vi "Dialog_TGC (SubVI).vi"() -> ()   [LabVIEW 2017]
uses:
  Control_EU/AScanXY.ctl
  Global_SNK3_HF.vi
panel:
  out "Array":dbl[](array[numeric])
  out "output array":dbl[](array[numeric])
  in  "Tab Control":T1(tab)
  out "DACTbl":dbl[][](array[numeric])
  out "TGC_Tbl":dbl[][](array[numeric])
  out "TGCTbl":dbl[][](array[numeric])=[[7.843137254901963e-08, 1.0457516339869285e-06, 2.1960784313725495e-06, 3.2941176470588244e-06, 4.078431372549021e-06, 4.993464052287583e-06, 5.725490196078433e-06, 7.686274509803923e-06, 8e-06], [0.039867986798679866, 0.030858085808580876, 0.036006600660066, 0.032574257425742575, 0.03900990099009902, 0.039438943894389455, 0.0282838283828383, 0.023993399339933996, 8e-06], [0.0, 1e-06, 2e-06, 3e-06, 4e-06, 5e-06, 6e-06, 7e-06, 8e-06], [0.0, 1e-06, 2e-06, 3e-06, 4e-06, 5e-06, 6e-06, 7e-06, 8e-06], [0.0, 1e-06, 2e-06, 3e-06, 4e-06, 5e-06, 6e-06, 7e-06, 8e-06], [0.0, 1e-06, 2e-06, 3e-06, 4e-06, 5e-06, 6e-06, 7e-06, 8e-06], [0.0, 1e-06, 2e-06, 3e-06, 4e-06, 5e-06, 6e-06, 7e-06, 8e-06], [0.0, 1e-06, 2e-06, 3e-06, 4e-06, 5e-06, 6e-06, 7e-06, 8e-06]]
  out "CurTbl":dbl[][](array[numeric])=[[7.843137254901963e-08, 1.0457516339869285e-06, 2.1960784313725495e-06, 3.2941176470588244e-06, 4.078431372549021e-06, 4.993464052287583e-06, 5.725490196078433e-06, 7.686274509803923e-06, 8e-06], [0.039867986798679866, 0.030858085808580876, 0.036006600660066, 0.032574257425742575, 0.03900990099009902, 0.039438943894389455, 0.0282838283828383, 0.023993399339933996, 8e-06], [0.0, 1e-06, 2e-06, 3e-06, 4e-06, 5e-06, 6e-06, 7e-06, 8e-06], [0.0, 1e-06, 2e-06, 3e-06, 4e-06, 5e-06, 6e-06, 7e-06, 8e-06], [0.0, 1e-06, 2e-06, 3e-06, 4e-06, 5e-06, 6e-06, 7e-06, 8e-06], [0.0, 1e-06, 2e-06, 3e-06, 4e-06, 5e-06, 6e-06, 7e-06, 8e-06], [0.0, 1e-06, 2e-06, 3e-06, 4e-06, 5e-06, 6e-06, 7e-06, 8e-06], [0.0, 1e-06, 2e-06, 3e-06, 4e-06, 5e-06, 6e-06, 7e-06, 8e-06]]
  in  "y":dbl=64.0 format="%#_13g"
  in  "Log":refnum<vi>
  in  "WrtTGC":bool
  in  "Tick":T2(ring)
  in  "ВРЧ":string[][](table)
  in  "Stop":bool
  out "TGCGraph":T3 caption="XY Graph - Light"
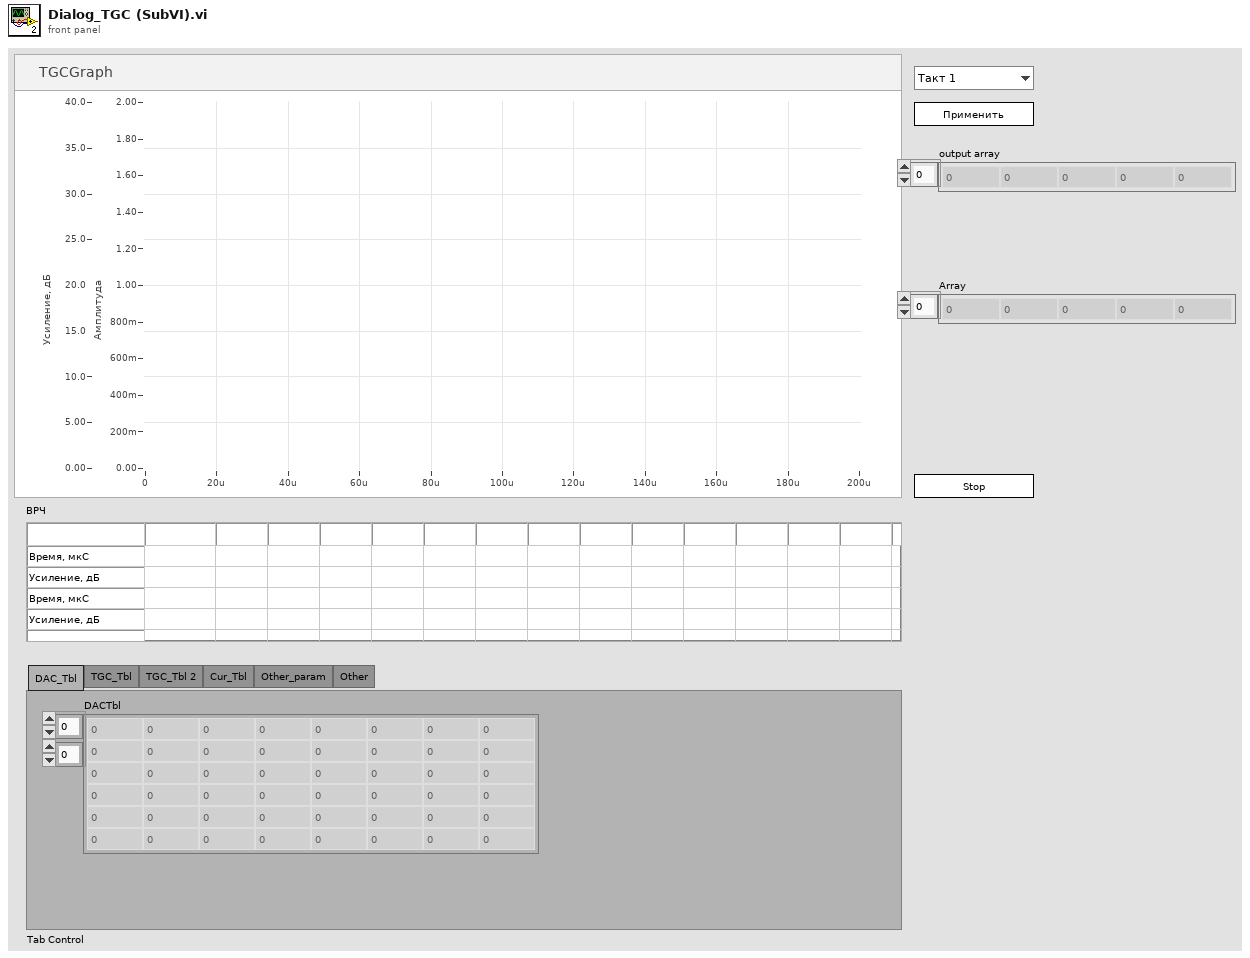
[diagram p1: front panel]
types:
  T1 = enum32{"DAC_Tbl", "TGC_Tbl", "TGC_Tbl 2", "Cur_Tbl", "Other_param", "Other"}
  T2 = enum16{"Такт 1", "Такт 2", "Такт 3", "Такт 4", "Такт 5", "Такт 6", "Такт 7", "Такт 8", "Такт 9", "Такт 10", "Такт 11", "Такт 12", "Такт 13", "Такт 14", "Такт 15", "Такт 16", "Такт 17", "Такт 18", "Такт 19", "Такт 20", "Такт 21", "Такт 22", "Такт 23", "Такт 24", "Такт 25", "Такт 26", "Такт 27", "Такт 28", "Такт 29", "Такт 30", "Такт 31", "Такт 32"}
  T3 = typedef "AScanXY.ctl" = cluster{dbl[], dbl[]}[]
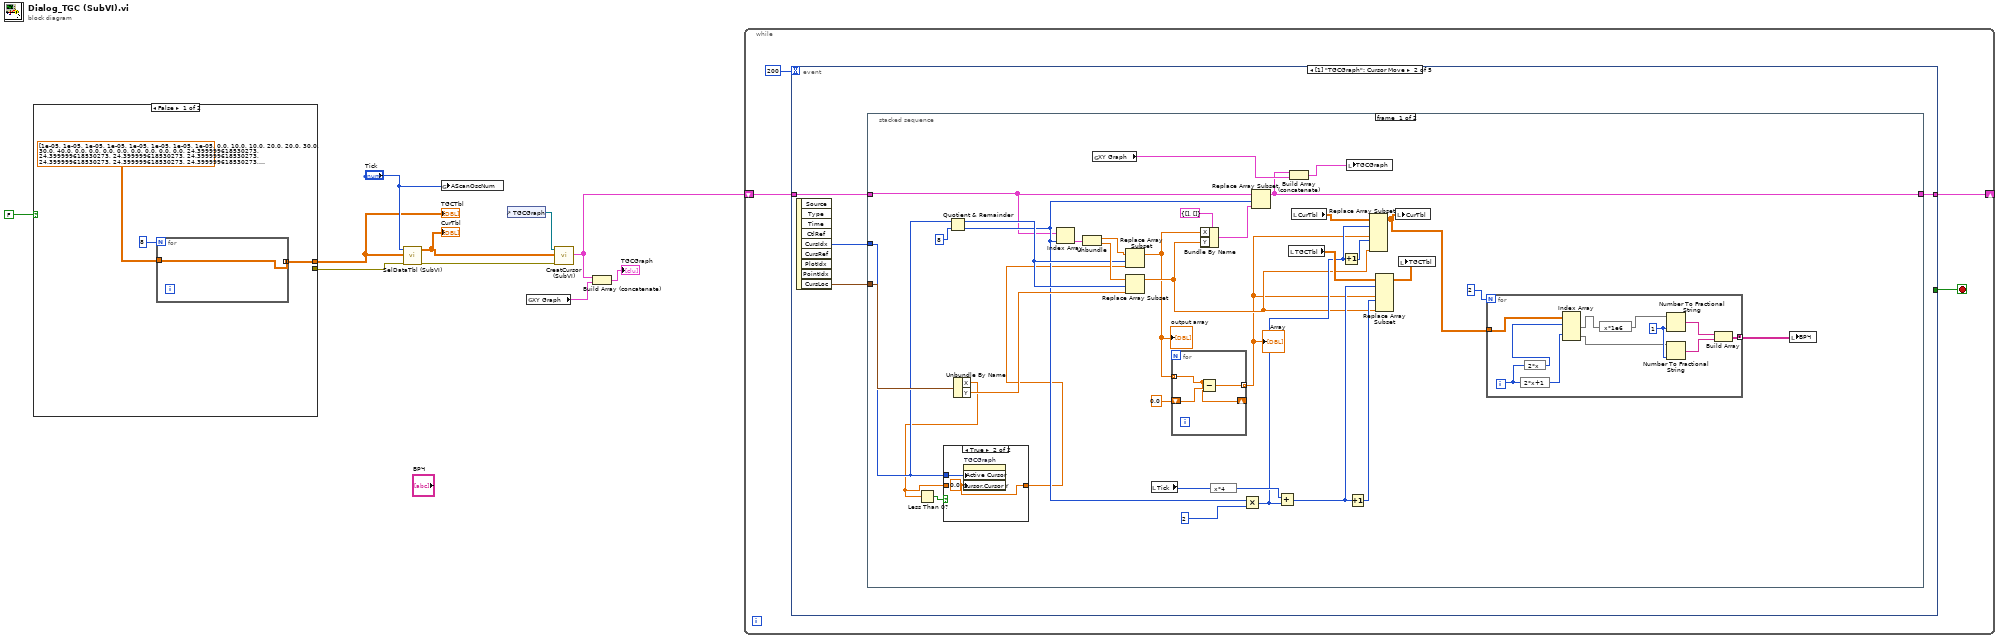
[diagram p0: block diagram]
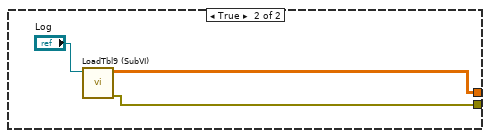
[diagram p2: hidden frame]
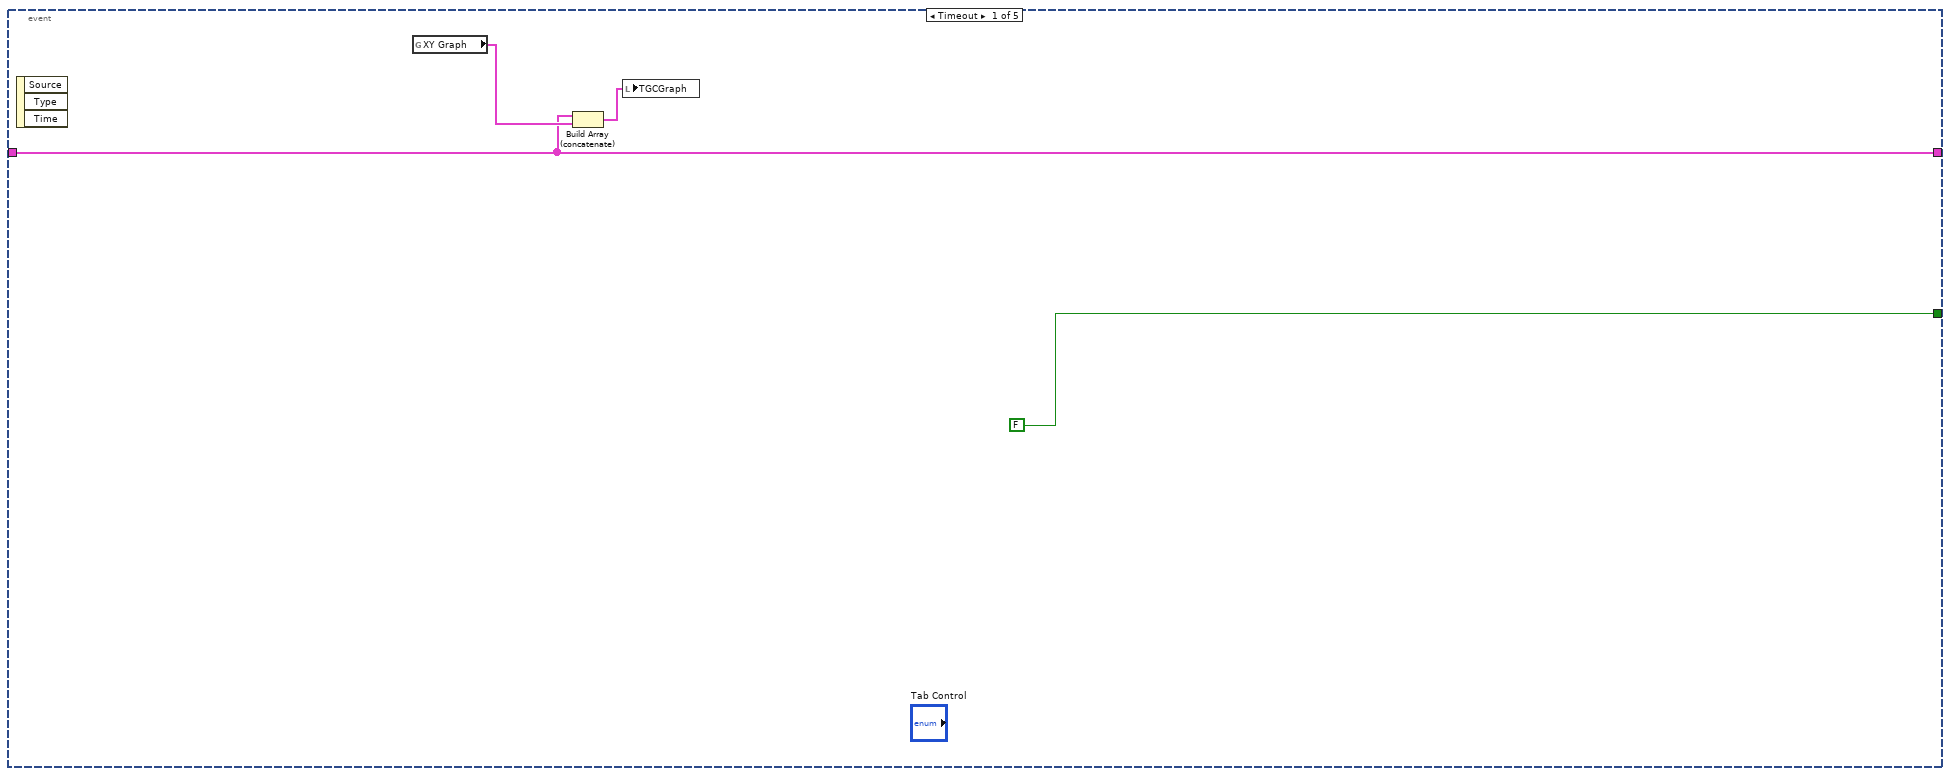
[diagram p3: hidden frame]
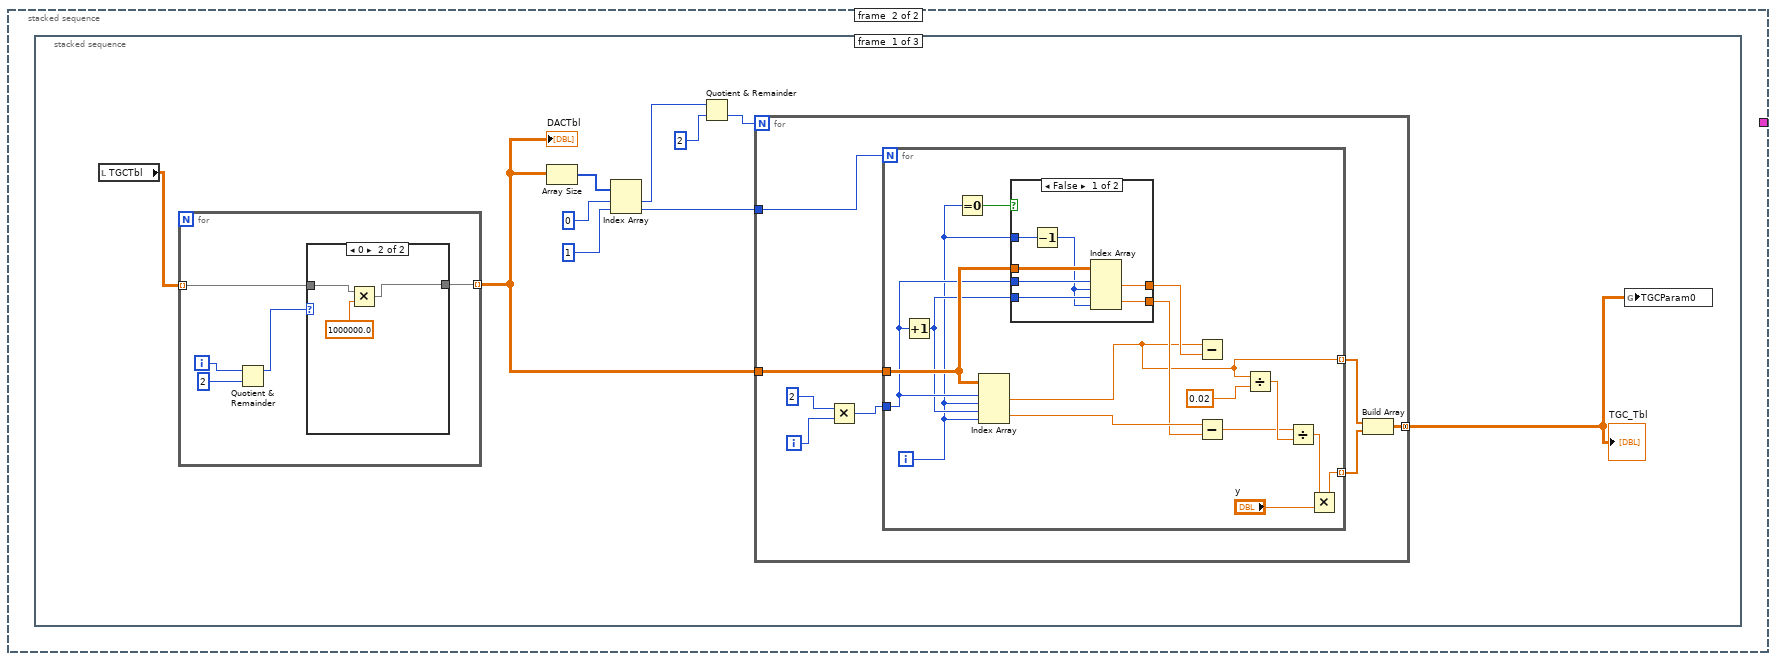
[diagram p5: hidden frame]
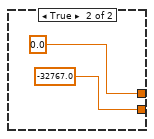
[diagram p6: hidden frame]
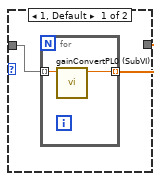
[diagram p7: hidden frame]
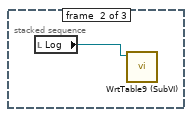
[diagram p8: hidden frame]
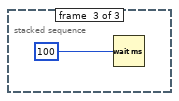
[diagram p9: hidden frame]
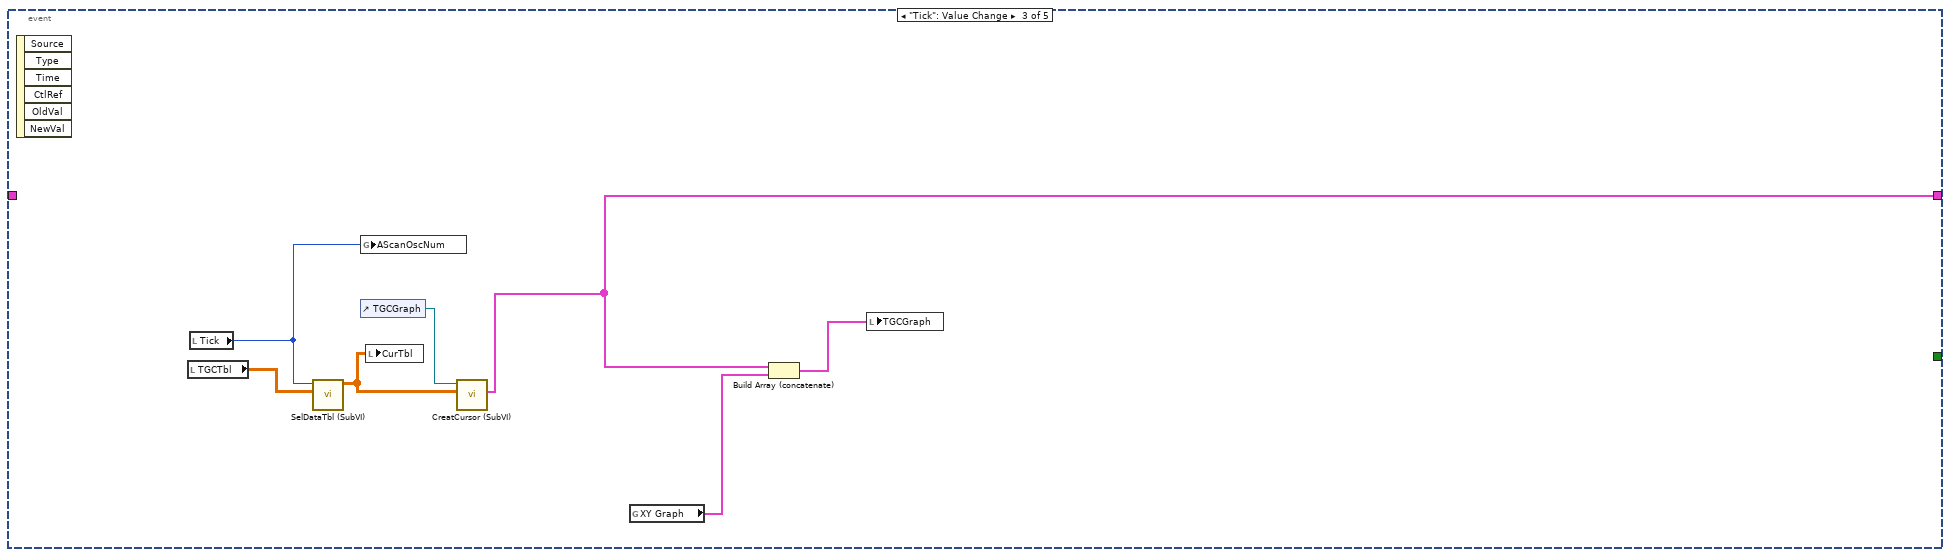
[diagram p10: hidden frame]
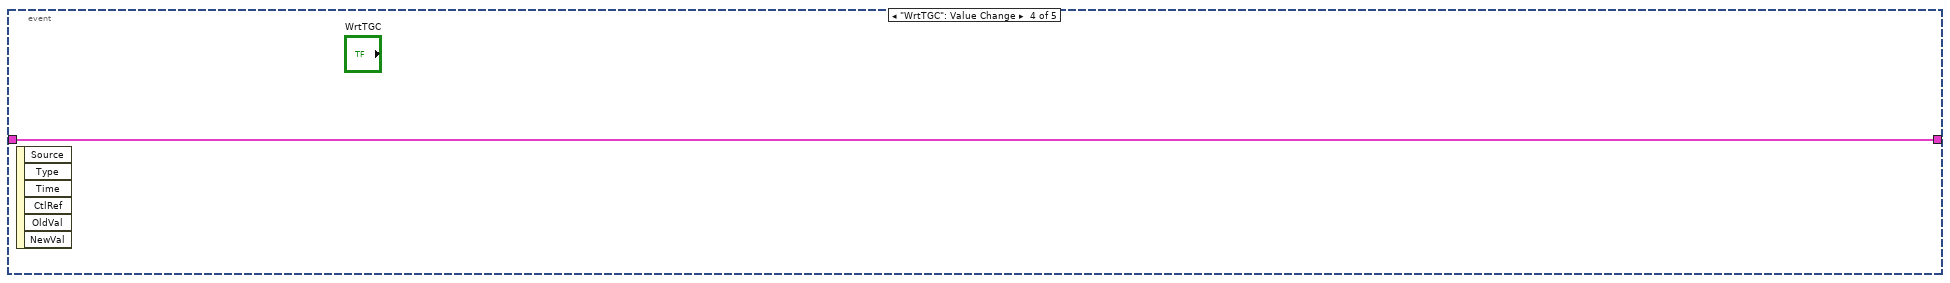
[diagram p11: hidden frame]
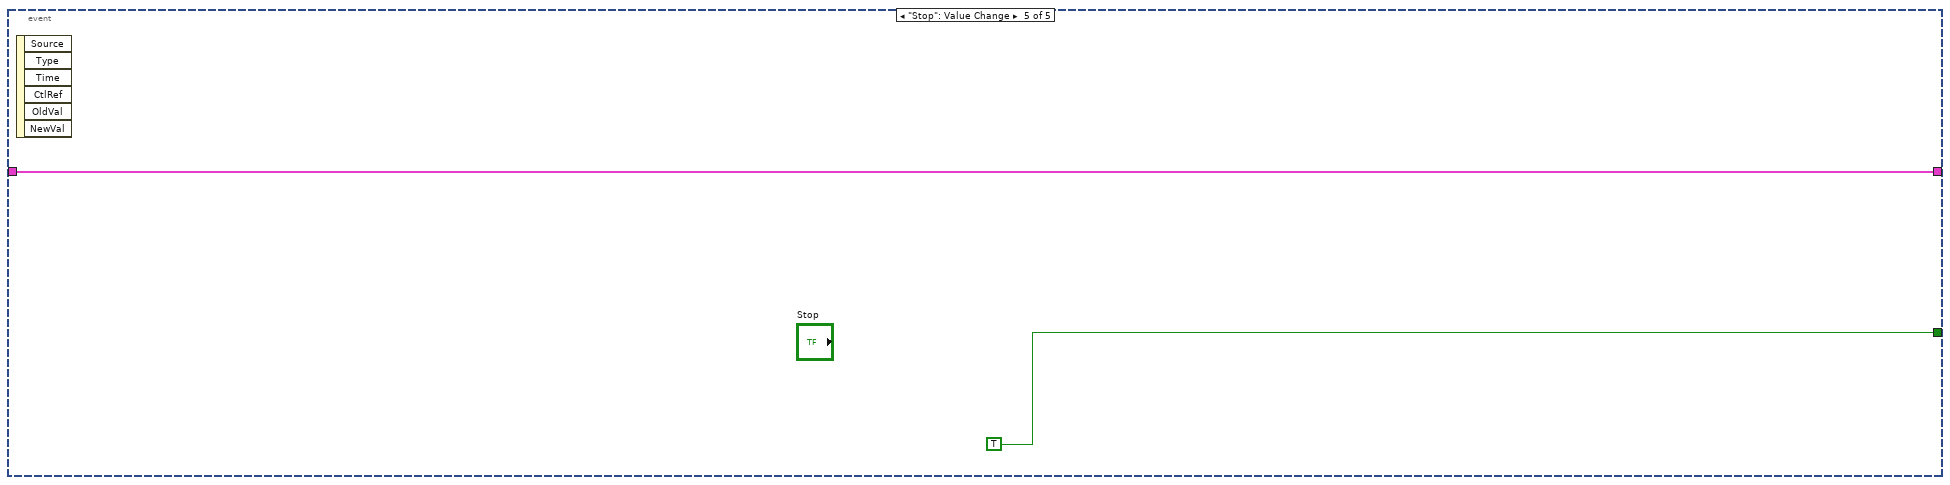
[diagram p12: hidden frame]
diagram:
  n1 = case shown="False" FALSE {
    tunnel: [w12 w16] -> w2
    tunnel: [_ w15] -> w1
    frame False {
      n2 = for {
        N: 8 -> [_]
        tunnel: [w14] -> w12 mode=concatenating
        tunnel: dbl[][] [[1e-05, 1e-05, 1e-05, 1e-05, 1e-05, 1e-05, 1e-05, 1e-05], [0.0, 10.0, 10.0, 20.0, 20.0, 30.0, 30.0, 40.0], [0.0, 0.0, 0.0, 0.0, 0.0, 0.0, 0.0, 0.0], [24.399999618530273, 24.399999618530273, 24.399999618530273, 24.399999618530273, 24.399999618530273, 24.399999618530273, 24.399999618530273, 24.399999618530273]] ("CurTbl 2") -> [w14]
      }
    }
    frame True {
      n3 = call "LoadTbl9 (SubVI).vi"("Log"="Log") -> ("error out"=w15:errorcluster, "Array"=w16:sgl[][])  [unwired: 9 in]
    }
  }
  "TGCTbl" <- w2
  n4 = call "SelDataTbl (SubVI).vi"("error in (no error)"=w1, "In"=w2, "Enum"="Tick") -> ("error out"=w4:errorcluster, "Out"=w3:dbl[][])  [unwired: 7 in]
  "CurTbl" <- w3
  n5 = global write "Global_SNK3_HF.vi" "AScanOscNum"("Tick") -> ()
  n6 = control-ref of="TGCGraph"() -> (w7:refnum<vi>)
  n7 = global read "Global_SNK3_HF.vi" "XY Graph"() -> (w10:cluster{dbl[], dbl[]})
  n8 = call "CreatCursor (SubVI).vi"("error in (no error)"=w4, "Array in"=w3, "XYGraph in"=w7) -> ("Array out"=w8:cluster{"X":dbl[], "Y":dbl[]}[])  [unwired: 8 in]
  n9 = Build Array (concatenate)(w8, w10) -> (→"TGCGraph":cluster{"X":dbl[], "Y":dbl[]}[])
  n10 = while {
    shift-right: [w19] -> _
    shift-left: w8 -> [w18]
    stop <- w21 stop-if-true
    n11 = event shown="[1] \"TGCGraph\": Cursor Move" {
      selector: _ -> [_ _ _ _ _]
      dyn-events: _ -> [_ _ _ _ _]
      timeout: 200 -> [_ _ _ _ _]
      tunnel: [FALSE _ _ _ TRUE] -> w21
      tunnel: w18 -> [w22 w27 _ w145 w146]
      tunnel: [w22 w28 w139 w145 w146] -> w19
      event Timeout {
        n12 = event-data() -> ()  [unwired: 1 in, 3 out]
        n13 = global read "Global_SNK3_HF.vi" "XY Graph"() -> (w24:cluster{dbl[], dbl[]})
        n14 = Build Array (concatenate)(w22, w24) -> (w23:cluster{"X":dbl[], "Y":dbl[]}[])
        n15 = local write "TGCGraph"(w23) -> ()
      }
      event Cursor Move {
        n16 = event-data() -> ("CursIdx"=w26:i32, "CursLoc"=w29:cluster{"X":dbl, "Y":dbl})  [unwired: 1 in, 7 out]
        n17 = stacked-sequence {
          tunnel: w29 -> [w64 _]
          tunnel: [w50 _] -> w28
          tunnel: w27 -> [w49 _]
          tunnel: w26 -> [w47 _]
          frame #0 {
            n18 = Quotient & Remainder(x=w47, y=8) -> (x-y*floor(x/y)=w55:i32, floor(x/y)=w53:i32)
            n19 = Unbundle By Name(w64) -> ("X"=w45:dbl, "Y"=w63:dbl)
            n20 = Less Than 0?(x=w45) -> (x < 0?=w46:bool)
            n21 = case shown="True" w46 {
              tunnel: w47 -> [_ w81]
              tunnel: w45 -> [w79 _]
              tunnel: [w79 w80] -> w44
              frame False {
              }
              frame True {
                w80 = 0.0 ("Cursor.Cursor Position:Cursor Y")
                n22 = property on="TGCGraph" class="XYGraph (strict)"("Active Cursor"=w81, "Cursor.Cursor Y"=w80) -> ()  [unwired: 2 in, 2 out]
              }
            }
            n23 = Index Array(array=w49, index=w53) -> (element=w60:cluster{"X":dbl[], "Y":dbl[]})
            n24 = Unbundle(w60) -> ("X"=w59:dbl[], "Y"=w58:dbl[])
            n25 = global read "Global_SNK3_HF.vi" "XY Graph"() -> (w52:cluster{dbl[], dbl[]})
            n26 = Replace Array Subset(array=w59, new element=w44, index=w55) -> (w32:dbl[])
            "output array" <- w32
            n27 = Replace Array Subset(array=w58, new element=w63, index=w55) -> (w36:dbl[])
            n28 = local read "Tick"() -> (w41:T2)
            n29 = for {
              tunnel: w32 -> [w65] mode=indexing
              tunnel: [w67] -> w30 mode=indexing
              shift-right: [w65] -> _
              shift-left: 0.0 -> [w66]
              n30 = Subtract(x=w65, y=w66) -> (x-y=w67:dbl)
            }
            "Array" <- w30
            n31 = Bundle By Name(cluster=cluster{"X":dbl[], "Y":dbl[]} {"X"=[], "Y"=[]}, "X"=w32, "Y"=w36) -> (w62:cluster{"X":dbl[], "Y":dbl[]})
            n32 = expression code="x*4"(w41) -> (w40:T2)
            n33 = Multiply(x=w53, y=2) -> (x*y=w38:i32)
            n34 = Replace Array Subset(array=w49, new element=w62, index=w53) -> (w50:cluster{"X":dbl[], "Y":dbl[]}[])
            n35 = Add(x=w40, y=w38) -> (x+y=w42:i32)
            n36 = local read "TGCTbl"() -> (w57:dbl[][])
            n37 = Build Array (concatenate)(w50, w52) -> (w51:cluster{"X":dbl[], "Y":dbl[]}[])
            n38 = local read "CurTbl"() -> (w39:dbl[][])
            n39 = Increment(x=w38) -> (x+1=w37:i32)
            n40 = local write "TGCGraph"(w51) -> ()
            n41 = Increment(x=w42) -> (x+1=w48:i32)
            n42 = Replace Array Subset(array=w39, new element #1=w30, index (row) #1=w38, new element #2=w36, index (row) #2=w37) -> (w34:dbl[][])  [unwired: 2 in]
            n43 = Replace Array Subset(array=w57, new element #1=w30, index (row) #1=w42, new element #2=w36, index (row) #2=w48) -> (w56:dbl[][])  [unwired: 2 in]
            n44 = local write "CurTbl"(w34) -> ()
            n45 = local write "TGCTbl"(w56) -> ()
            n46 = for {
              N: 2 -> [_]
              tunnel: w34 -> [w75]
              tunnel: [w71] -> w33 mode=concatenating
              i -> [w74]
              w76 = i16 1 ("precision (6)")
              n47 = expression code="2*x+1"(w74) -> (w72:i32)
              n48 = expression code="2*x"(w74) -> (w73:i32)
              n49 = Index Array(array=w75, index (row) #1=w73, index (row) #2=w72) -> (element #1=w69:dbl[], element #2=w70:dbl[])  [unwired: 2 in]
              n50 = expression code="x*1e6"(w69) -> (w68:dbl[])
              n51 = Number To Fractional String(number=w68, precision (6)=w76) -> (F-format string=w78:string[])  [unwired: 2 in]
              n52 = Number To Fractional String(number=w70, precision (6)=w76) -> (F-format string=w77:string[])  [unwired: 2 in]
              n53 = Build Array(w78, w77) -> (w71:string[][])
            }
            n54 = local write "ВРЧ"(w33) -> ()
          }
          frame #1 {
            n55 = stacked-sequence {
              frame #0 {
                n56 = local read "TGCTbl"() -> (w91:dbl[][])
                n57 = for {
                  tunnel: w91 -> [w125] mode=indexing
                  tunnel: [w124] -> w83 mode=indexing
                  i -> [w128]
                  n58 = Quotient & Remainder(x=w128, y=2) -> (x-y*floor(x/y)=w126:i32)  [unwired: 1 out]
                  n59 = case shown="0" w126 {
                    tunnel: w125 -> [w130 w135]
                    tunnel: [w129 w134] -> w124
                    frame 1, Default {
                      n60 = for {
                        tunnel: w130 -> [w132] mode=indexing
                        tunnel: [w131] -> w129 mode=indexing
                        n61 = call "gainConvertPL0 (SubVI).vi"("GainIN"=w132) -> ("DACout"=w131:dbl)  [unwired: 8 in, 2 out]
                      }
                    }
                    frame 0 {
                      n62 = Multiply(x=w135, y=1000000.0) -> (x*y=w134:dbl[])
                    }
                  }
                }
                "DACTbl" <- w83
                n63 = Array Size(array=w83) -> (size(s)=w90:i32[])
                n64 = Index Array(array=w90, index #1=0 ("index"), index #2=1 ("index")) -> (element #1=w87:i32, element #2=w84:i32)
                n65 = Quotient & Remainder(x=w87, y=2) -> (floor(x/y)=w88:i32)  [unwired: 1 out]
                n66 = for {
                  N: w88 -> [_]
                  tunnel: w84 -> [w99]
                  tunnel: w83 -> [w98]
                  tunnel: [w92] -> w82 mode=concatenating
                  i -> [w95]
                  n67 = Multiply(x=2, y=w95) -> (x*y=w96:i32)
                  n68 = for {
                    N: w99 -> [_]
                    tunnel: w98 -> [w114]
                    tunnel: w96 -> [w113]
                    tunnel: [w102] -> w93 mode=indexing
                    tunnel: [w100] -> w94 mode=indexing
                    i -> [w104]
                    n69 = Increment(x=w113) -> (x+1=w112:i32)
                    n70 = Equal To 0?(x=w104) -> (x = 0?=w105:bool)
                    n71 = Index Array(array=w114, index (row) #1=w113, index (col) #1=w104, index (row) #2=w112, index (col) #2=w104) -> (element #1=w100:dbl, element #2=w110:dbl)
                    n72 = case shown="False" w105 {
                      tunnel: w114 -> [w121 _]
                      tunnel: w113 -> [w117 _]
                      tunnel: w112 -> [w116 _]
                      tunnel: w104 -> [w120 _]
                      tunnel: [w119 0.0 ("DACout")] -> w111
                      tunnel: [w118 -32767.0 ("DACout")] -> w109
                      frame False {
                        n73 = Decrement(x=w120) -> (x-1=w115:i32)
                        n74 = Index Array(array=w121, index (row) #1=w117, index (col) #1=w115, index (row) #2=w116, index (col) #2=w115) -> (element #1=w119:dbl, element #2=w118:dbl)
                      }
                      frame True {
                      }
                    }
                    n75 = Subtract(x=w100, y=w111) -> ()  [unwired: 1 out]
                    n76 = Subtract(x=w110, y=w109) -> (x-y=w106:dbl)
                    n77 = Divide(x=w100, y=0.02) -> (x/y=w107:dbl)
                    n78 = Divide(x=w106, y=w107) -> (x/y=w103:dbl)
                    n79 = Multiply(x=w103, y="y") -> (x*y=w102:dbl)
                  }
                  n80 = Build Array(w94, w93) -> (w92:dbl[][])
                }
                "TGC_Tbl" <- w82
                n81 = global write "Global_SNK3_HF.vi" "TGCParam0"(w82) -> ()
              }
              frame #1 {
                n82 = local read "Log"() -> (w136:refnum<vi>)
                n83 = call "WrtTable9 (SubVI).vi"("Log"=w136) -> ()  [unwired: 10 in, 1 out]
              }
              frame #2 {
                n84 = Wait (ms)(milliseconds to wait=u32 100) -> ()  [unwired: 1 out]
              }
            }
          }
        }
      }
      event "Tick": Value Change {
        n85 = event-data() -> ()  [unwired: 1 in, 6 out]
        n86 = local read "TGCTbl"() -> (w143:dbl[][])
        n87 = local read "Tick"() -> (w138:T2)
        n88 = call "SelDataTbl (SubVI).vi"("In"=w143, "Enum"=w138) -> ("Out"=w144:dbl[][])  [unwired: 8 in, 1 out]
        n89 = global write "Global_SNK3_HF.vi" "AScanOscNum"(w138) -> ()
        n90 = control-ref of="TGCGraph"() -> (w142:refnum<vi>)
        n91 = local write "CurTbl"(w144) -> ()
        n92 = call "CreatCursor (SubVI).vi"("Array in"=w144, "XYGraph in"=w142) -> ("Array out"=w139:cluster{"X":dbl[], "Y":dbl[]}[])  [unwired: 9 in]
        n93 = global read "Global_SNK3_HF.vi" "XY Graph"() -> (w141:cluster{dbl[], dbl[]})
        n94 = Build Array (concatenate)(w139, w141) -> (w140:cluster{"X":dbl[], "Y":dbl[]}[])
        n95 = local write "TGCGraph"(w140) -> ()
      }
      event "WrtTGC": Value Change {
        n96 = event-data() -> ()  [unwired: 1 in, 6 out]
      }
      event "Stop": Value Change {
        n97 = event-data() -> ()  [unwired: 1 in, 6 out]
      }
    }
  }
